vi "Init Events.vi"(8 "error in (no error)":errorcluster, 11 "DeviceListPanel in":refnum<class "DeviceListPanel.lvclass">) -> (0 "error out":errorcluster, 3 "DeviceListPanel out":refnum<class "DeviceListPanel.lvclass">)   [LabVIEW 2020, in "PicoG-App.lvlib" / "DeviceListPanel.lvclass"]
uses:
  DeviceListPanel.lvclass
  Device/Device Key.ctl
  Device/Device.lvclass
  DeviceListPanel.lvclass/DeviceListPanel.ctl
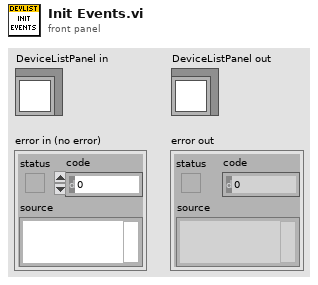
[diagram p1: front panel]
types:
  T1 = typedef "PicoG-App.lvlib/Device.lvclass/Device Key.ctl" = cluster{"Platform":string, "Board":string, "ID":string}
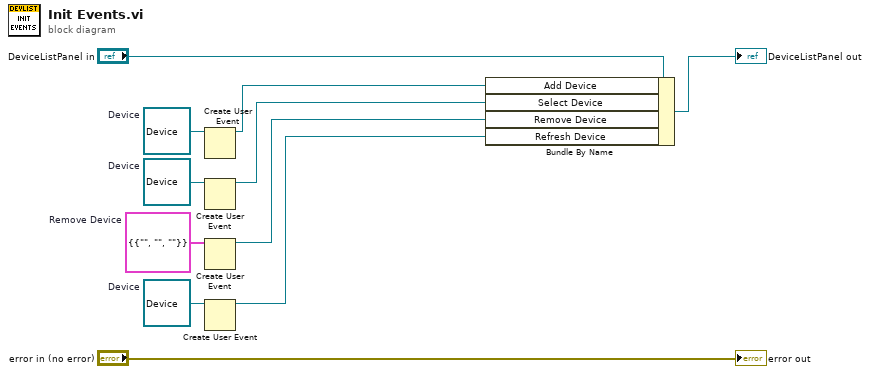
[diagram p0: block diagram]
diagram:
  w2 = refnum<class "Device.lvclass"> refnum  # Device
  w4 = cluster{"Device Key":T1} {"Device Key"={"Platform"="", "Board"="", "ID"=""}}  # Remove Device
  w6 = refnum<class "Device.lvclass"> refnum  # Device
  w10 = refnum<class "Device.lvclass"> refnum  # Device
  n1 = Create User Event(user event datatype=w10) -> (user event=w9:refnum<user-event>)  [unwired: 1 in, 1 out]
  n2 = Create User Event(user event datatype=w6) -> (user event=w5:refnum<user-event>)  [unwired: 1 in, 1 out]
  n3 = Create User Event(user event datatype=w4) -> (user event=w3:refnum<user-event>)  [unwired: 1 in, 1 out]
  n4 = Create User Event(user event datatype=w2) -> (user event=w1:refnum<user-event>)  [unwired: 1 in, 1 out]
  n5 = Bundle By Name(cluster="DeviceListPanel in", "Add Device"=w9, "Select Device"=w5, "Remove Device"=w3, "Refresh Device"=w1) -> (→"DeviceListPanel out":refnum<class "DeviceListPanel.lvclass">)
  "error out" <- "error in (no error)"
